vi "Sample.vi"(8 "错误输入（无错误）":errorcluster, 10 "基本信息":T1={"USB Port"="", "采集间隔(s)"=0.5, "坐标选择"=enum."X", "Axis"=["X", "Y", "Z", "T"], "Unit"=["X", "Y", "Z", "T"]}) -> (0 "错误输出":errorcluster, 2 "PoNSp":dbl[](array[numeric]))   [LabVIEW 2026, in "UI-Zolix.lvlib" / "Acquisition.lvlib"]
uses:
  Acquisition.lvlib
  Supports/Sample Settings.ctl
  UI-Zolix.lvlib
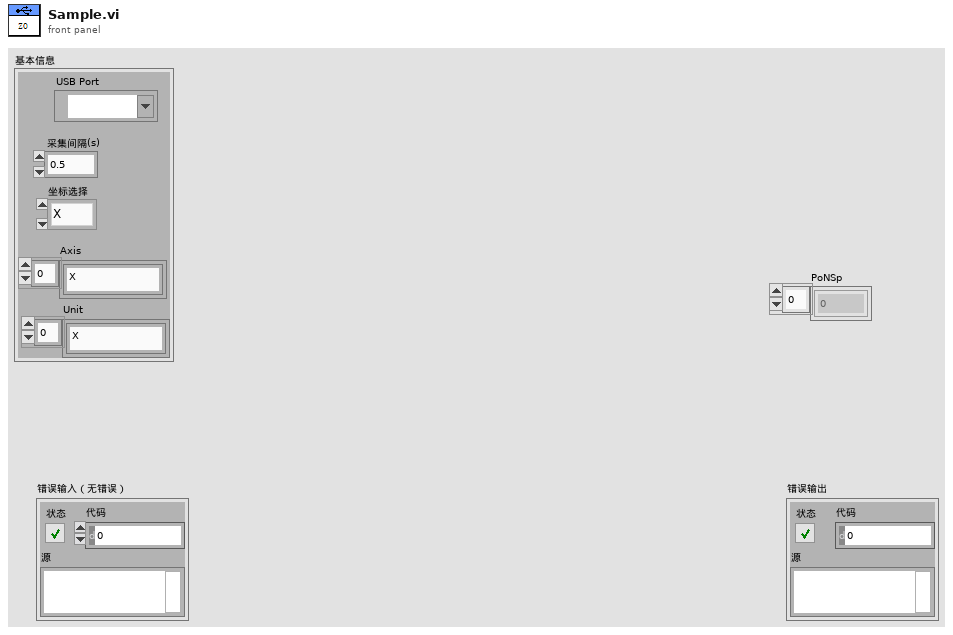
[diagram p1: front panel]
types:
  T1 = typedef "UI-Zolix.lvlib/Sample Settings.ctl" = cluster{"USB Port":refnum<visa-resource-name>, "采集间隔(s)":dbl, "坐标选择":enum32{"X", "Y", "Z", "T"}, "Axis":string[], "Unit":string[]}
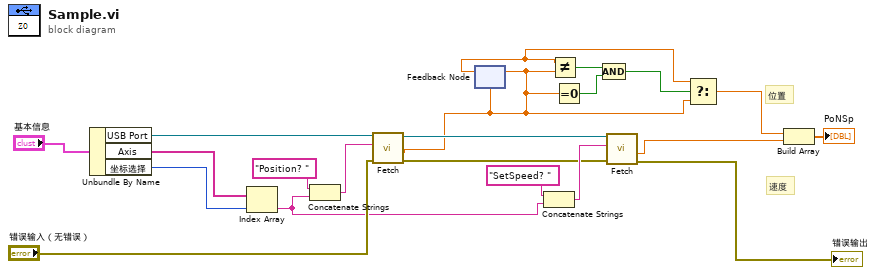
[diagram p0: block diagram]
diagram:
  # "速度"
  # "位置"
  n1 = Unbundle By Name("基本信息") -> ("USB Port"=w14:refnum<visa-resource-name>, "Axis"=w17:string[], "坐标选择"=w15:enum32{"X", "Y", "Z", "T"})
  n2 = Index Array(array=w17, index=w15) -> (element=w8:string)
  n3 = Concatenate Strings("Position? ", w8) -> (w18:string)
  n4 = call "Fetch.vi"("错误输入"="错误输入（无错误）", "Command"=w18, "VISA资源"=w14) -> ("错误输出"=w7:errorcluster, "数值"=w2:dbl, "VISA资源"=w11:refnum<visa-resource-name>)  [unwired: 3 in, 3 out]
  n5 = feedback #1(w2) -> (w3:dbl)
  n6 = feedback-in #1(w2) -> ()
  n7 = Concatenate Strings("SetSpeed? ", w8) -> (w13:string)
  n8 = Not Equal?(x=w3, y=w2) -> (x != y?=w6:bool)
  n9 = Equal To 0?(x=w2) -> (x = 0?=w5:bool)
  n10 = Compound Arithmetic op=AND ("复合运算")(w6, w5) -> (w4:bool)
  n11 = call "Fetch.vi"("错误输入"=w7, "Command"=w13, "VISA资源"=w11) -> ("错误输出"=→"错误输出":errorcluster, "数值"=w9:dbl)  [unwired: 3 in, 4 out]
  n12 = Select(t=w3, s=w4, f=w2) -> (s? t:f=w1:dbl)
  n13 = Build Array(w1, w9) -> (→"PoNSp":dbl[])
